vi "5.vi"() -> ()   [LabVIEW 2013]
panel:
  out "Voltage":dbl
  out "Voltage":dbl(knob) scale=0.0..230.0
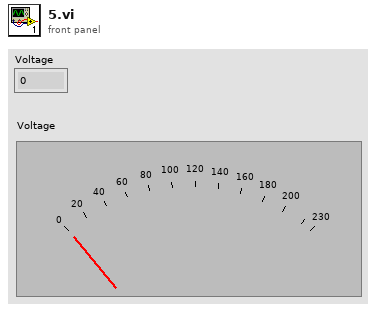
[diagram p1: front panel]
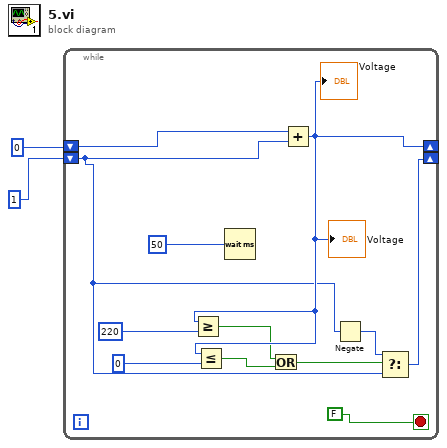
[diagram p0: block diagram]
diagram:
  n1 = while {
    shift-right: [w10] -> _
    shift-left: 0 -> [w13]
    shift-right: [w5] -> _
    shift-left: 1 -> [w4]
    stop <- FALSE stop-if-true
    n2 = Wait (ms)(milliseconds to wait=50) -> ()  [unwired: 1 out]
    n3 = Add(x=w13, y=w4) -> (x+y=w10:i32)
    "Voltage" <- w10
    "Voltage" <- w10
    n4 = Greater Or Equal?(x=w10, y=220) -> (x >= y?=w9:bool)
    n5 = Less Or Equal?(x=w10, y=0) -> (x <= y?=w8:bool)
    n6 = Or(x=w9, y=w8) -> (x .or. y?=w7:bool)
    n7 = Negate(x=w4) -> (-x=w6:i32)
    n8 = Select(t=w6, s=w7, f=w4) -> (s? t:f=w5:i32)
  }
